vi "acc-daq-test.vi"() -> ()   [LabVIEW 2026, in "Unit-Test.lvlib"]
uses:
  Unit-Test.lvlib
  src/Vibration-Core/Calculations.lvlib
  <vilib>/DAQmx/configure/timing.llb/DAQmx Timing (Sample Clock).vi
  <vilib>/DAQmx/read.llb/DAQmx Read (Analog 1D Wfm NChan NSamp).vi
  <vilib>/DAQmx/create/channels.llb/DAQmx Create Channel (AI-Acceleration-Accelerometer).vi
  <vilib>/addons/_NISVFA/_Shared subVIs/Controls/svc_Window.ctl
panel:
  in  "window":T1=1 items=["None"=0, "Hanning"=1, "Hamming"=2, "Blackman-Harris"=3, "Exact Blackman"=4, "Blackman"=5, "Flat Top"=6, "4 Term B-Harris "=7, "7 Term B-Harris"=8, "Low Sidelobe"=9, "Force"=64, "Exponential"=65, "Blackman Nuttall"=11, "Triangle"=30, "Bartlett-Hanning"=31, "Bohman"=32, "Parzen"=33, "Welch"=34, "Kaiser"=60, "Dolph-Chebyshev"=61, "Gaussian"=62]
  out "Waveform Graph":waveform(dbl)[](graph)
  in  "stop":bool
  out "Meas array":dbl[][](array[numeric])
  out "Array":waveform(dbl)[](array[waveform])
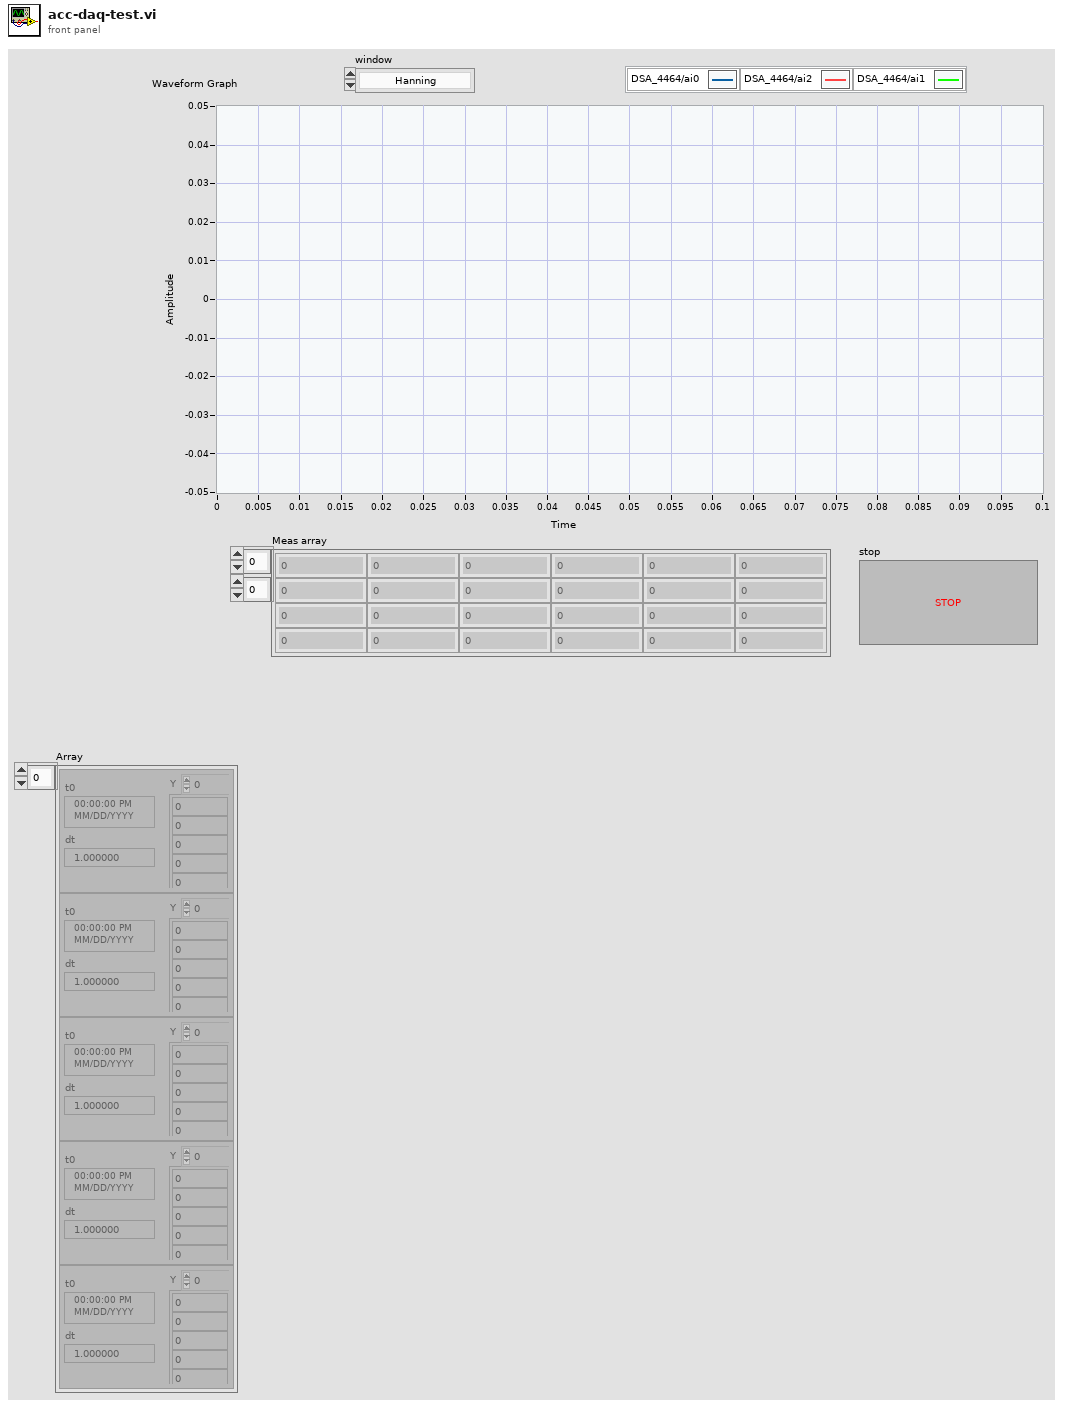
[diagram p1: front panel]
types:
  T1 = typedef "svc_Window.ctl" = u32
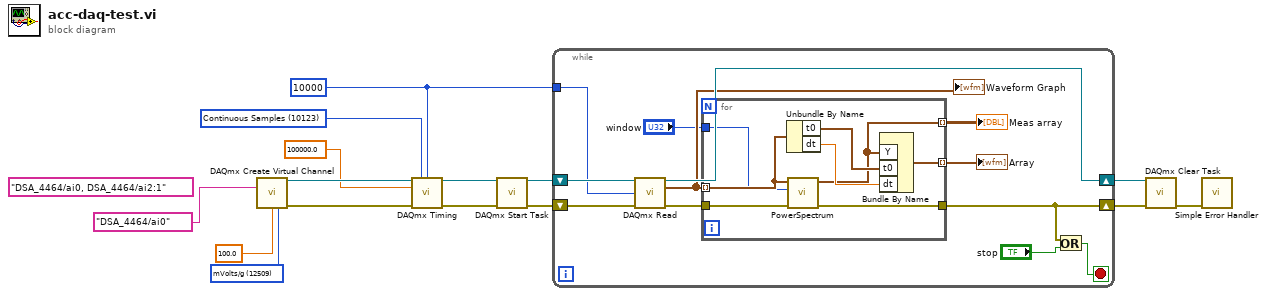
[diagram p0: block diagram]
diagram:
  w3 = 12509 items=["mVolts/g"=12509, "Volts/g"=12510] ("sensitivity units")
  w4 = 10000 ("samples per channel")
  w6 = 10123 items=["Finite Samples"=10178, "Continuous Samples"=10123, "Hardware Timed Single Point"=12522] ("sample mode")
  (unwired) tag "DSA_4464/ai0, DSA_4464/ai2:1" ("physical channels")
  n1 = call-poly <vilib>:"DAQmx Create Virtual Channel.vi"("physical channels"=tag "DSA_4464/ai0", "sensitivity"=100.0, "sensitivity units"=w3) -> ("task out"=w7:refnum<k21>, "error out"=w8:errorcluster)  [unwired: 11 in]
  n2 = call-poly <vilib>:"DAQmx Timing.vi"("task/channels in"=w7, "sample mode"=w6, "samples per channel"=w4, "rate"=100000.0, "error in"=w8) -> ("task out"=w10:refnum<k21>, "error out"=w9:errorcluster)  [unwired: 9 in]
  n3 = call <vilib>:"DAQmx Start Task.vi"("task/channels in"=w10, "error in"=w9) -> ("task out"=w13:refnum<k21>, "error out"=w12:errorcluster)  [unwired: 12 in]
  n4 = while {
    shift-right: [w26] -> w14
    shift-left: w13 -> [w25]
    shift-right: [w19] -> w15
    shift-left: w12 -> [w24]
    tunnel: w4 -> [w21]
    stop <- w17 stop-if-true
    n5 = call-poly <vilib>:"DAQmx Read.vi"("task/channels in"=w25, "number of samples per channel"=w21, "error in"=w24) -> ("task out"=w26:refnum<k21>, "data"=w20:waveform(dbl)[], "error out"=w23:errorcluster)  [unwired: 10 in]
    "Waveform Graph" <- w20
    n6 = for {
      tunnel: w20 -> [w30] mode=indexing
      tunnel: w23 -> [w35]
      tunnel: [w34] -> w19
      tunnel: [w33] -> w27 mode=indexing
      tunnel: [w29] -> w22 mode=indexing
      tunnel: "window" -> [w28]
      n7 = Unbundle By Name(w30) -> ("t0"=w32:timestamp, "dt"=w31:dbl)
      n8 = call "PowerSpectrum.vi"("error in (no error)"=w35, "Window"=w28, "Data In"=w30) -> ("error out"=w34:errorcluster, "Array of Waveforms"=w29:waveform(dbl)[])  [unwired: 6 in, 1 out]
      n9 = Bundle By Name("Y"=w29, "t0"=w32, "dt"=w31) -> (w33:waveform(dbl))  [unwired: 1 in]
    }
    "Array" <- w27
    "Meas array" <- w22
    n10 = Or(x=w19, y="stop") -> (x .or. y?=w17:bool)
  }
  n11 = call <vilib>:"DAQmx Clear Task.vi"("task in"=w14, "error in"=w15) -> ("error out"=w11:errorcluster)  [unwired: 13 in]
  n12 = call <vilib>:"Simple Error Handler.vi"("error in (no error)"=w11) -> ()  [unwired: 4 in, 5 out]
